vi "Read DAQ FIFO.vi"(8 "error in (no error)":errorcluster, 9 "Timeout (ms)":i32, 10 "Data In":T1[](array[typedef]), 11 "CIFFIFO in":refnum<class "CIF_Iceoryx_Fifo_DAQ.lvclass">) -> (0 "error out":errorcluster, 1 "timed out?":bool, 2 "Data Out":T1[](array[typedef]), 3 "CIFFIFO out":refnum<class "CIF_Iceoryx_Fifo_DAQ.lvclass">, 4 "Header":T2)   [LabVIEW 2021, in "CIF_Iceoryx_Fifo_DAQ.lvclass"]
uses:
  CIF_Iceoryx_Fifo_DAQ.lvclass
  ChannelCommon/typedef/FIFO Header.ctl
  D:/dev/Packages/CIF_Channels_Core/src/Iceorxy_Channels/PCAP_Universal/CIF_Iceoryx_PCAP_Universal.lvclass
  D:/dev/Packages/CIF_Channels_Core/src/CIFChannels/CIFChannels.lvclass
  ChannelCommon/typedef/Datatype Waveform.ctl
  CIFChannels/CIFChannels.lvclass/CIFChannels.ctl
  PCAP_Universal/CIF_Iceoryx_PCAP_Universal.lvclass/CIF_Iceoryx_PCAP_Universal.ctl
  <vilib>/CIF Foundation/CIF Utilities/Statistics/I64/Stats_I64_CIF_U.lvclass/Stats_I64_CIF_U.ctl
  <vilib>/CIF Foundation/CIF Utilities/DataTypes/Typedef/Endian.ctl
  <vilib>/CIF Foundation/CIF PCAP Parse and Build/pcap_Parse_Build_CIF.lvclass
  <vilib>/CIF Foundation/CIF PCAP Parse and Build/pcap_Parse_Build_CIF.lvclass/pcap_Parse_Build_CIF.ctl
  28377979-7082-45c0-88da-dd60acddcbb6.vi
  ff34c1be-f7c8-4825-89bb-b930973add4f.vi
  4225e33e-6553-49b2-86d3-1a9e3dd855c7.vi
  CIFChannels/Accessors/Read FIFO Header.vi
  PCAP_Universal/Accessors/Read Payload.vi
  <vilib>/CIF Foundation/CIF PCAP Parse and Build/Data Accessors/Write OS Endian.vi
  <vilib>/CIF Foundation/CIF PCAP Parse and Build/Parse/Unflatten Packet Header.vi
  28377979-7082-45c0-88da-dd60acddcbb6.vi/c28b0ead-42ad-4072-80a2-aca7f2bd7ce3.vi
  28377979-7082-45c0-88da-dd60acddcbb6.vi/48104490-ec73-4168-8754-ff252ec03617.vi
  <vilib>/CIF Foundation/CIF Utilities/DataTypes/SubVIs/DataTypes Error.vi
  28377979-7082-45c0-88da-dd60acddcbb6.vi/a935433e-9fba-46a4-a99d-56703b8e2dfe.vi
  <vilib>/CIF Foundation/CIF Utilities/Time/System Time/Get System Time.vi
  <vilib>/CIF Foundation/CIF Utilities/Statistics/I64/X1 minus X0.vi
  PCAP_Universal/Accessors/Read CIF Subscriber Refnum.vi
  <vilib>/CIF Foundation/CIF Iceoryx/PubSub/CIF pcap/CIF Receive.vi
  ChannelCommon/Utilities/Remove Header Bytes.vi
  CIFChannels/Accessors/Write FIFO Header.vi
  CIFChannels/Utilities/Update Channel Benchmark.vi
  PCAP_Universal/SubVIs/Core Read U8 FIFO.vi/e703c505-0034-46a9-8989-21c0de27793f.vi
  PCAP_Universal/SubVIs/Core Read U8 FIFO.vi/768488f4-e6df-4560-a449-a64b33b49031.vi
  CIFChannels/Accessors/Read Channel State.vi
  CIFChannels/Accessors/Read Direction.vi
  <vilib>/CIF Foundation/CIF PCAP Parse and Build/Utilities/Add Error.vi
  <vilib>/CIF Foundation/CIF Utilities/DataTypes/Flatten Unflatten/Unflatten U32.vi
  <vilib>/CIF Foundation/CIF Utilities/Statistics/I64/X1 minus X0.vi/dfabcf33-0dbc-4041-80a5-3dc0c86d2989.vi
  <vilib>/CIF Foundation/CIF Iceoryx/SubVIs/Get Path.vi
  <vilib>/CIF Foundation/CIF Iceoryx/SubVIs/Convert Error.vi
  <vilib>/CIF Foundation/CIF Iceoryx/Refnum/CIF Subscriber from Refnum.vi
  <vilib>/CIF Foundation/CIF Utilities/Statistics/I64/X1 minus X0.vi/dfabcf33-0dbc-4041-80a5-3dc0c86d2989.vi/9eb60a9a-770f-4d2d-8b3f-8465c267ecc9.vi
  PCAP_Universal/CIF_Iceoryx_PCAP_Universal.lvclass
  <vilib>/CIF Foundation/CIF Iceoryx/SubVIs/Convert Error Core.vi
  <vilib>/CIF Foundation/CIF PCAP Parse and Build/Utilities/Add Error Core.vi
  <vilib>/CIF Foundation/CIF Utilities/DataTypes/SubVIs/DataTypes Error Core.vi
  CIF_Iceoryx_Fifo_DAQ.lvclass/CIF_Iceoryx_Fifo_DAQ.ctl
  <vilib>/CIF Foundation/CIF PCAP DAQ/PCAP DAQ Core.lvlib
  <vilib>/CIF Foundation/CIF Utilities/DataTypes/DataTypes_CIF_U.lvlib
  CIFChannels/CIFChannels.lvclass
  ChannelCommon/ChannelCommon.lvlib
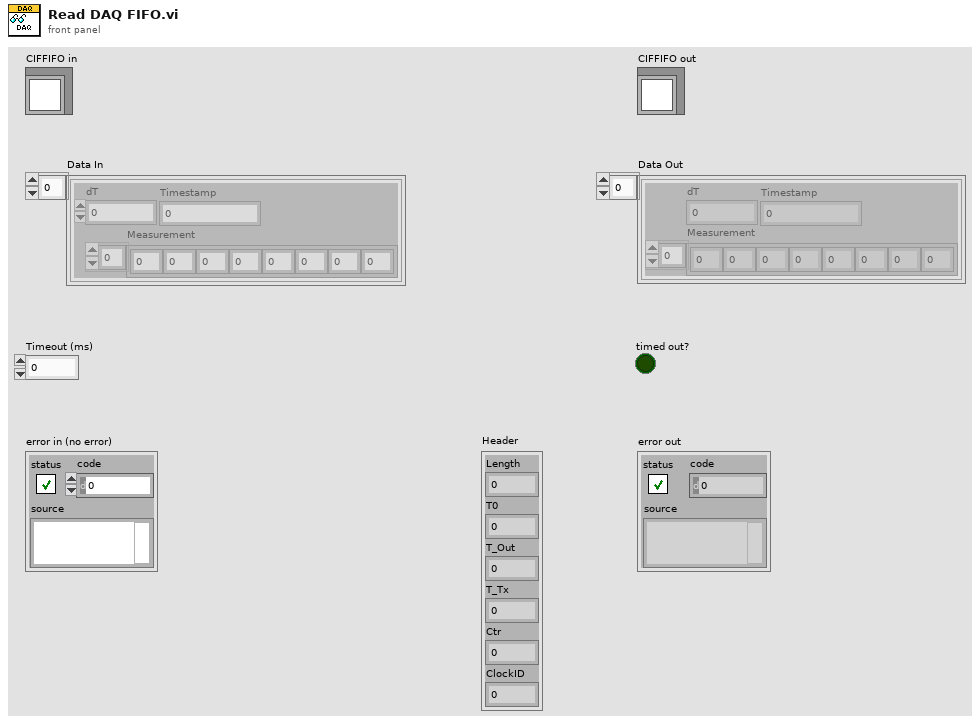
[diagram p1: front panel]
types:
  T1 = typedef "ChannelCommon.lvlib/Datatype Waveform.ctl" = cluster{"Measurement":dbl[], "dT":dbl, "Timestamp":i64}
  T2 = typedef "ChannelCommon.lvlib/FIFO Header.ctl" = cluster{"Length":u64, "T0":i64, "T_Out":i64, "T_Tx":i64, "Ctr":u64, "ClockID":u8}
  T3 = typedef "DataTypes_CIF_U.lvlib/Endian.ctl" = enum16{"Little Endian", "Big Endian"}
  T4 = typedef "PCAP DAQ Core.lvlib/DAQ Header.ctl" = cluster{"dT (s)":dbl, "Channels":u16, "Endian":enum16{"Little Endian", "Big Endian"}, "Interleaved":T5}
  T5 = typedef "PCAP DAQ Core.lvlib/Interleaved.ctl" = enum8{"Concatenated", "Interleaved"}
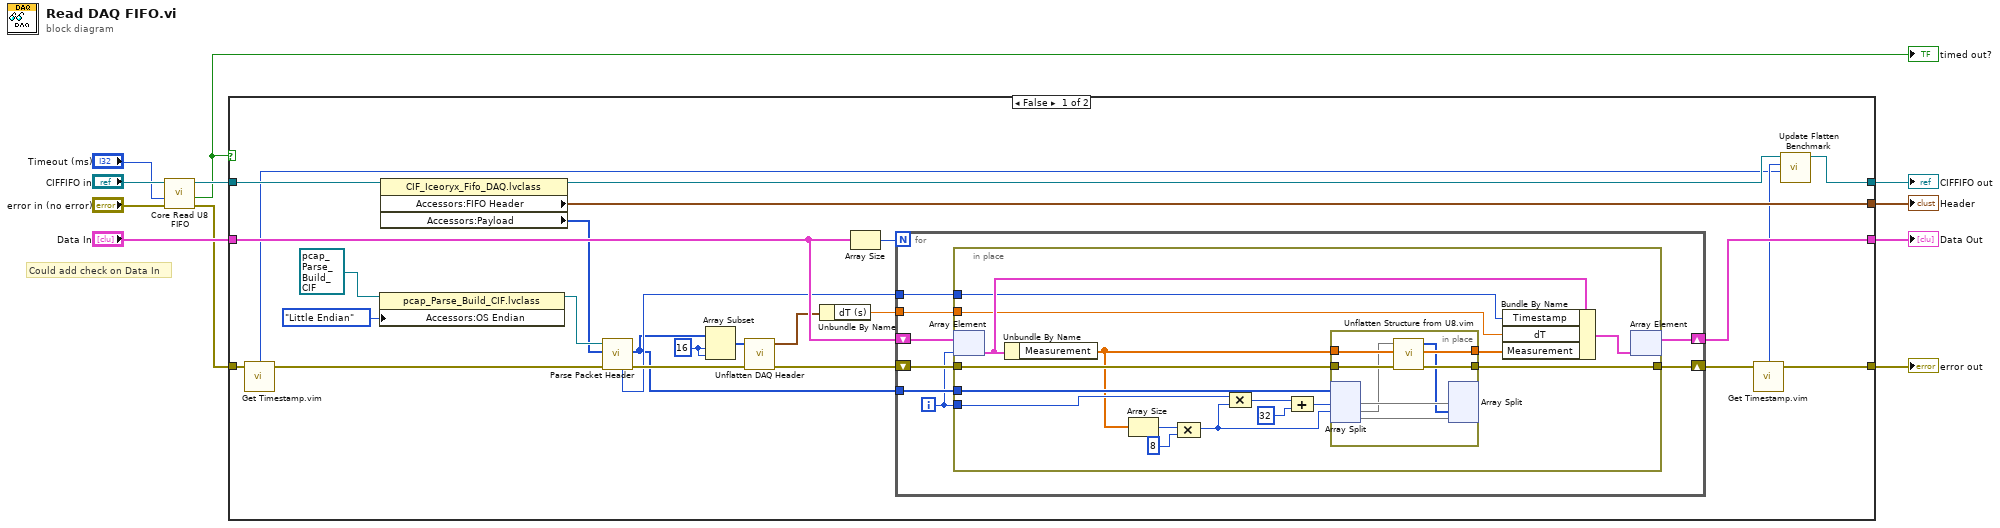
[diagram p0: block diagram]
diagram:
  # "Could add check on Data In"
  n1 = call "Core Read U8 FIFO.vi"("error in (no error)"="error in (no error)", "Timeout (ms)"="Timeout (ms)", "CIFFIFO in"="CIFFIFO in") -> ("error out"=w6:errorcluster, "timed out?"=w2:bool, "CIFFIFO out"=w4:refnum<class "CIF_Iceoryx_Fifo_DAQ.lvclass">)  [unwired: 6 in]
  "timed out?" <- w2
  n2 = case shown="False" w2 {
    tunnel: w4 -> [w14 w69]
    tunnel: [w23 w71] -> w9
    tunnel: [w36 _] -> w11
    tunnel: "Data In" -> [w26 w71]
    tunnel: w6 -> [w20 w70]
    tunnel: [w17 w70] -> w5
    tunnel: [w15 w69] -> w3
    frame False {
      w32 = 16 ("index")
      n3 = call "Get Timestamp.vim"("Anything in"=w20) -> ("Time (ns)"=w12:i64, "Anything out"=w19:errorcluster)  [unwired: 2 in]
      n4 = property class="pcap_Parse_Build_CIF.lvclass"(reference=refnum<class "pcap_Parse_Build_CIF.lvclass"> refnum ("pcap Parse and Build in"), "Accessors:OS Endian"=Endian."Little Endian" ("OS Endian")) -> (reference out=w33:refnum<class "pcap_Parse_Build_CIF.lvclass">)  [unwired: 1 in, 1 out]
      n5 = property class="CIF_Iceoryx_Fifo_DAQ.lvclass"(reference=w14) -> (reference out=w16:refnum<class "CIF_Iceoryx_Fifo_DAQ.lvclass">, "Accessors:FIFO Header"=w36:T2, "Accessors:Payload"=w21:u8[])  [unwired: 1 in, 1 out]
      n6 = call <vilib>:"Parse Packet Header.vi"("error in (no error)"=w19, "Bytes in"=w21, "pcap Parse and Build in"=w33) -> ("error out"=w30:errorcluster, "Bytes out"=w22:u8[], "TAI Time (ns)"=w24:i64)  [unwired: 3 in, 3 out]
      n7 = Array Subset(array=w22, index=w32, length=w32) -> (w31:u8[])
      n8 = call <vilib>:"Unflatten DAQ Header.vi"("error in"=w30, "Flat DAQ Header"=w31) -> ("error out"=w29:errorcluster, "DAQ Header"=w25:T4)  [unwired: 8 in]
      n9 = Unbundle By Name(w25) -> ("dT (s)"=w27:dbl)
      n10 = Array Size(array=w26) -> (size(s)=w28:i32)
      n11 = for {
        N: w28 -> [_]
        tunnel: w22 -> [w44]
        shift-right: [w40] -> w18
        shift-left: w29 -> [w42]
        shift-right: [w37] -> w23
        shift-left: w26 -> [w43]
        tunnel: w27 -> [w39]
        tunnel: w24 -> [w38]
        i -> [w41]
        n12 = in-place {
          in-place-border: w44 -> [w60]
          in-place-border: w41 -> [w59]
          in-place-border: w42 -> [w57]
          in-place-border: [w53] -> w40
          in-place-border: w39 -> [w50]
          in-place-border: w38 -> [w49]
          n13 = in-place-array #1(w43, w41) -> (w56:T1)
          n14 = Unbundle By Name(w56) -> ("Measurement"=w45:dbl[])
          n15 = Array Size(array=w45) -> (size(s)=w47:i32)
          n16 = Compound Arithmetic op=MULTIPLY(w47, 8 ("value")) -> (w46:i32)
          n17 = Compound Arithmetic op=MULTIPLY(w59, w46) -> (w52:i32)
          n18 = Compound Arithmetic op=ADD(w52, 32 ("value")) -> (w58:i32)
          n19 = in-place {
            in-place-border: w45 -> [w66]
            in-place-border: w57 -> [w65]
            in-place-border: [w64] -> w55
            in-place-border: [w63] -> w53
            n20 = in-place-split #2(w60, w58, w46) -> (w68:u8[], w62:u8[], w67:u8[])
            n21 = call "Unflatten Structure from U8.vim"("error in"=w65, "Type"=w66, "Flattend Data in"=w62) -> ("error out"=w63:errorcluster, "Unflattend Data"=w64:dbl[], "Flatten Data out"=w61:u8[])  [unwired: 6 in]
            n22 = in-place-split #2(w68, w61, w67) -> ()  [unwired: 3 out]
          }
          n23 = Bundle By Name(cluster=w56, "Timestamp"=w49, "dT"=w50, "Measurement"=w55) -> (w54:T1)
          n24 = in-place-array #1(w54) -> (w37:T1[])  [unwired: 1 out]
        }
      }
      n25 = call "Get Timestamp.vim"("Anything in"=w18) -> ("Time (ns)"=w13:i64, "Anything out"=w17:errorcluster)  [unwired: 2 in]
      n26 = call "Update Flatten Benchmark.vi"("X0"=w12, "X1"=w13, "CIFChannels in"=w16) -> ("CIFChannels out"=w15:refnum<class "CIF_Iceoryx_Fifo_DAQ.lvclass">)  [unwired: 7 in, 1 out]
    }
    frame True {
    }
  }
  "error out" <- w5
  "Header" <- w11
  "CIFFIFO out" <- w3
  "Data Out" <- w9
